vi "VIH Dialog - VI Terminals - Shortcut Menu Handler - Tree.vi"(6 "Menu Tag":string, 9 "MenuRef":refnum<k9>, 10 "Terminals Tree":refnum<vi>, 11 "Event Type":T1) -> (3 "States spec":string)   [LabVIEW 2014]
doc: "::: VI Helpeks :::\nCopyright (c) 2000-2026 Konstantin Shifershteyn. All rights reserved."
uses:
  <vilib>/event_ctls.llb/lveventtype.ctl
  <vilib>/Utility/miscctls.llb/LVNodeAndColumnTypeDef.ctl
  _VIH Support Library.llb/VIH Utility - MENU - Create Menu (String).vi
panel:
  # "VI Helpeks\nCopyright (c) 2012-2026 Konstantin Shifershteyn"
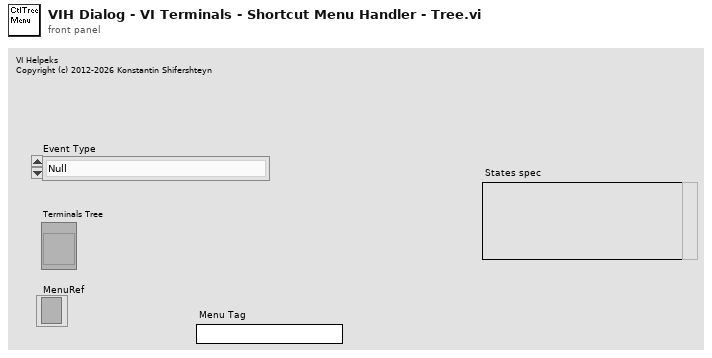
[diagram p1: front panel]
types:
  T1 = typedef "lveventtype.ctl" = enum32{"Null", "Timeout", "Annotation Menu Selection", "Annotation Menu Selection?", "App Instance Close", "App Instance Close?", "Autoscale Range Change", "Bookmark Info Change", "Cell Edit", "Cell Edit?", "Cursor Grab", "Cursor Grab?", "Cursor Menu Selection", "Cursor Menu Selection?", "Cursor Move", "Cursor Release", "Data Change", "Direction Change", "Display State Change", "Drag Ended", "Drag Enter", "Drag Leave", "Drag Over", "Drag Source Update", "Drag Starting", "Drag Starting?", "Drop", "Exec State Change", "Key Down", "Key Down?", "Key Repeat", "Key Repeat?", "Key Up", "Listbox Double Click", "Menu Activation?", "Menu Selection (App)", "Menu Selection? (App)", "Menu Selection (User)", "Mouse Down", "Mouse Down?", "Mouse Enter", "Mouse Leave", "Mouse Move", "Mouse Up", "Mouse Wheel", "NI Security User Change (App)", "Pane Size", "Panel Close", "Panel Close?", "Panel Resize", "Plot Attribute Change", "Scale Range Change", "Shortcut Menu Activation?", "Shortcut Menu Selection (App)", "Shortcut Menu Selection? (App)", "Shortcut Menu Selection (User)", "Tree Double Click", "Tree Drag", "Tree Drag?", "Tree Drop", "Tree Drop?", "Tree Item Close", "Tree Item Close?", "Tree Item Open", "Tree Item Open?", "User Event", "Value Change"}
  T2 = typedef "LVNodeAndColumnTypeDef.ctl" = cluster{"Node":string, "Column":i32}
  T3 = typedef "VIH Project Tree Typedef - Tree Refnum.ctl" = refnum<vi>
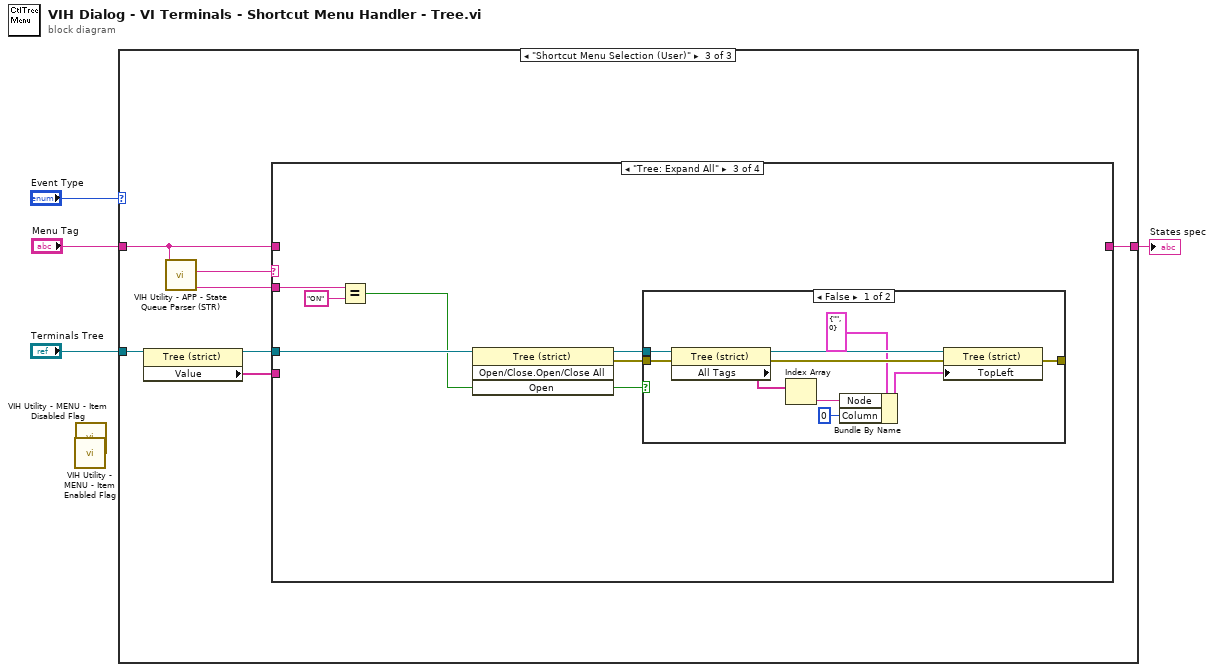
[diagram p0: block diagram]
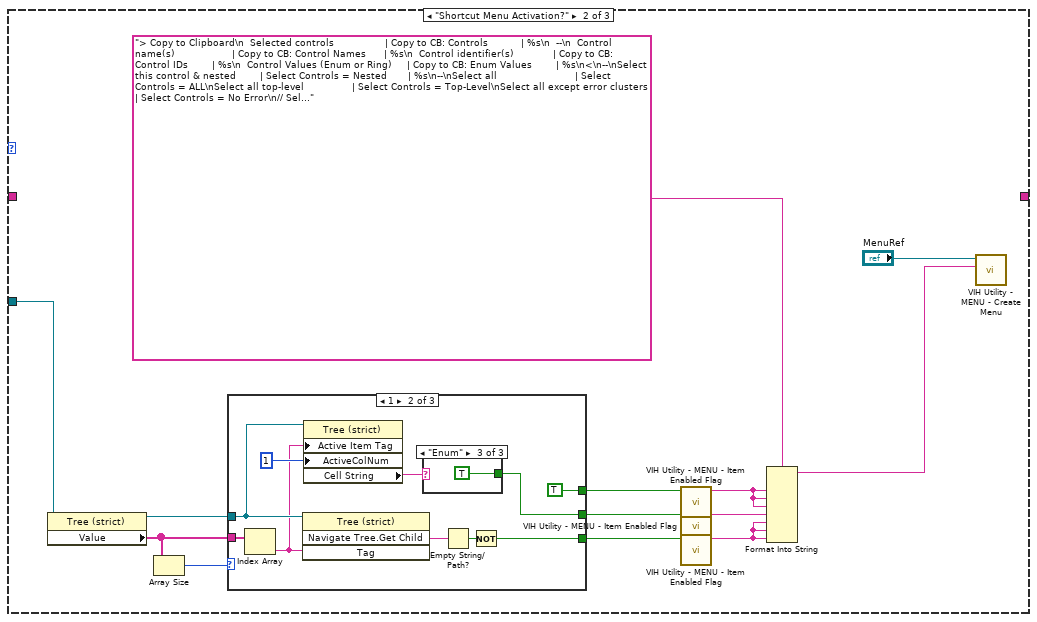
[diagram p3: hidden frame]
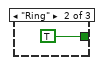
[diagram p6: hidden frame]
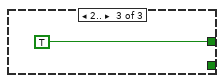
[diagram p7: hidden frame]
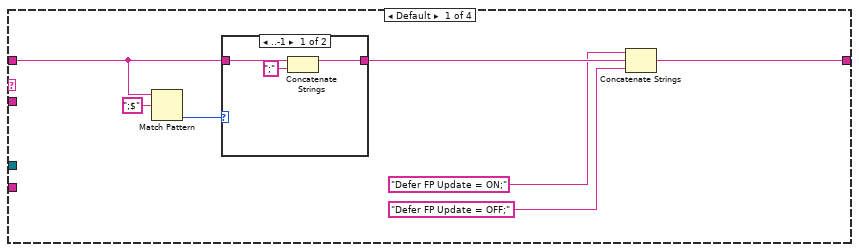
[diagram p8: hidden frame]
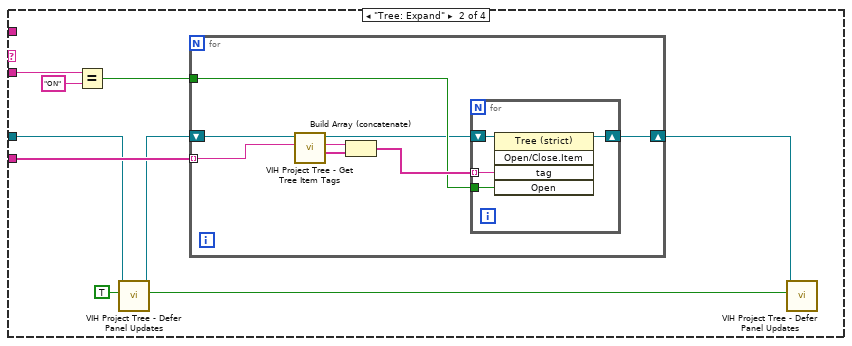
[diagram p10: hidden frame]
diagram:
  n1 = call "VIH Utility - MENU - Item Enabled Flag.vi"() -> ()  [unwired: 11 in, 1 out]
  n2 = call "VIH Utility - MENU - Item Disabled Flag.vi"() -> ()  [unwired: 11 in, 1 out]
  n3 = case shown="\"Shortcut Menu Selection (User)\"" "Event Type" {
    tunnel: "Terminals Tree" -> [_ w17 w34]
    tunnel: [_ _ w32] -> w2
    tunnel: "Menu Tag" -> [_ _ w36]
    frame Default {
    }
    frame "Shortcut Menu Activation?" {
      n4 = property class="Tree (strict)"(reference=w17) -> (reference out=w14:refnum<vi>, "Value"=w6:string[])  [unwired: 1 in, 1 out]
      n5 = Array Size(array=w6) -> (size(s)=w9:i32)
      n6 = case shown="1" w9 {
        tunnel: w14 -> [_ w22 _]
        tunnel: [_ w25 _] -> w8
        tunnel: w6 -> [_ w24 _]
        tunnel: [_ TRUE TRUE] -> w7
        tunnel: [_ w18 _] -> w5
        frame ..0 {
        }
        frame 1 {
          n7 = Index Array(array=w24) -> (element=w20:string)  [unwired: 1 in]
          n8 = invoke class="Tree (strict)" method="Navigate Tree.Get Child"(reference=w22, "Tag"=w20) -> ("Navigate Tree:Get Child"=w27:string)  [unwired: 2 in, 3 out]
          n9 = property class="Tree (strict)"(reference=w22, "Active Item Tag"=w20, "ActiveColNum"=1 ("Active Cell:Active Column Number")) -> ("Cell String"=w19:string)  [unwired: 1 in, 2 out]
          n10 = case shown="\"Enum\"" w19 {
            tunnel: [_ TRUE TRUE] -> w18
            frame Default {
            }
            frame "Ring" {
            }
            frame "Enum" {
            }
          }
          n11 = Empty String/Path?(string/path=w27) -> (empty?=w26:bool)
          n12 = Not(x=w26) -> (.not. x?=w25:bool)
        }
        frame 2.. {
        }
      }
      n13 = call "VIH Utility - MENU - Item Enabled Flag.vi"("Enable?"=w7) -> ("Disable flag"=w10:string)  [unwired: 10 in]
      n14 = call "VIH Utility - MENU - Item Enabled Flag.vi"("Enable?"=w5) -> ("Disable flag"=w11:string)  [unwired: 10 in]
      n15 = call "VIH Utility - MENU - Item Enabled Flag.vi"("Enable?"=w8) -> ("Disable flag"=w12:string)  [unwired: 10 in]
      n16 = Format Into String(format string="> Copy to Clipboard\n  Selected controls                 | Copy to CB: Controls           | %s\n  --\n  Control name(s)                   | Copy to CB: Control Names      | %s\n  Control identifier(s)             | Copy to CB: Control IDs        | %s\n  Control Values (Enum or Ring)     | Copy to CB: Enum Values        | %s\n<\n--\nSelect this control & nested        | Select Controls = Nested       | %s\n--\nSelect all                          | Select Controls = ALL\nSelect all top-level                | Select Controls = Top-Level\nSelect all except error clusters    | Select Controls = No Error\n// Select error clusters               | Select Controls = Error\nSelect Enum & Ring controls         | Select Controls = Enum & Ring\n--\n> Expand/Collapse Tree\n  Expand all                        | Tree: Expand All = ON\n  Collapse all                      | Tree: Expand All = OFF\n  --\n  Expand nested                     | Tree: Expand = ON              | %s\n  Collapse nested                   | Tree: Expand = OFF             | %s\n<", w10, w10, w10, w11, w12, w12, w12) -> (resulting string=w13:string)  [unwired: 2 in, 1 out]
      n17 = call-poly "VIH Utility - MENU - Create Menu.vi"("Menu Description"=w13, "menu"="MenuRef") -> ()  [unwired: 8 in, 2 out]
    }
    frame "Shortcut Menu Selection (User)" {
      n18 = property class="Tree (strict)"(reference=w34) -> (reference out=w33:refnum<vi>, "Value"=w35:string[])  [unwired: 1 in, 1 out]
      n19 = call "VIH Utility - APP - State Queue Parser (STR).vi"("input queue"=w36) -> ("state parameters"=w31:string, "state"=w37:string)  [unwired: 5 in, 2 out]
      n20 = case shown="\"Tree: Expand All\"" w37 {
        tunnel: [w40 _ _ _] -> w32
        tunnel: w36 -> [w42 _ _ _]
        tunnel: w33 -> [_ w54 w73 _]
        tunnel: w35 -> [_ w57 _ _]
        tunnel: w31 -> [_ w56 w75 _]
        frame Default {
          n21 = Match Pattern(string=w42, regular expression=";$") -> (offset past match=w43:i32)  [unwired: 1 in, 3 out]
          n22 = case shown="..-1" w43 {
            tunnel: w42 -> [w47 w48]
            tunnel: [w46 w48] -> w41
            frame ..-1 {
              n23 = Concatenate Strings(w47, ";" ("string")) -> (w46:string)
            }
            frame 0.. {
            }
          }
          n24 = Concatenate Strings("Defer FP Update = ON;", w41, "Defer FP Update = OFF;") -> (w40:string)
        }
        frame "Tree: Expand" {
          n25 = Equal?(x=w56, y="ON") -> (x = y?=w49:bool)
          n26 = call "VIH Project Tree - Defer Panel Updates.vi"("Defer Panel Updates (F)"=TRUE, "Project Tree"=w54) -> ("Previous Defer status"=w51:bool, "dup Project Tree"=w53:T3)  [unwired: 7 in, 1 out]
          n27 = for {
            tunnel: w57 -> [w62] mode=indexing
            shift-right: [w63] -> w52
            shift-left: w53 -> [w65]
            tunnel: w49 -> [w59]
            n28 = call "VIH Project Tree - Get Tree Item Tags.vi"("Parent Item Tag"=w62, "Project Tree"=w65) -> ("Child Item Tags"=w60:string[], "dup Parent Item Tag"=w61:string, "dup Project Tree"=w58:T3)  [unwired: 6 in, 1 out]
            n29 = Build Array (concatenate)(w61, w60) -> (w64:string[])
            n30 = for {
              tunnel: w64 -> [w68] mode=indexing
              tunnel: w59 -> [w67]
              shift-right: [w66] -> w63
              shift-left: w58 -> [w69]
              n31 = invoke class="Tree (strict)" method="Open/Close.Item"(reference=w69, "tag"=w68, "Open"=w67) -> (reference out=w66:T3)  [unwired: 2 in, 4 out]
            }
          }
          n32 = call "VIH Project Tree - Defer Panel Updates.vi"("Defer Panel Updates (F)"=w51, "Project Tree"=w52) -> ()  [unwired: 7 in, 3 out]
        }
        frame "Tree: Expand All" {
          n33 = Equal?(x=w75, y="ON") -> (x = y?=w70:bool)
          n34 = invoke class="Tree (strict)" method="Open/Close.Open/Close All"(reference=w73, "Open"=w70) -> (reference out=w72:refnum<vi>, error out=w71:errorcluster)  [unwired: 2 in, 2 out]
          n35 = case shown="False" w70 {
            tunnel: [w82 w86] -> _
            tunnel: w71 -> [w80 w86]
            tunnel: w72 -> [w79 _]
            frame False {
              n36 = property class="Tree (strict)"(reference=w79, error in=w80) -> (reference out=w78:refnum<vi>, error out=w81:errorcluster, "All Tags"=w85:string[])
              n37 = Index Array(array=w85) -> (element=w84:string)  [unwired: 1 in]
              n38 = Bundle By Name(cluster=T2 {"Node"="", "Column"=0} ("Top Left Visible Cell"), "Node"=w84, "Column"=0) -> (w76:T2)
              n39 = property class="Tree (strict)"(reference=w78, error in=w81, "TopLeft"=w76) -> (error out=w82:errorcluster)  [unwired: 1 out]
            }
            frame True {
            }
          }
        }
        frame "----------------------------- 1" {
        }
      }
    }
  }
  "States spec" <- w2
